vi "lua_monitor.vi"(11 "Lua for LabVIEW.lvlib:Lua.lvclass":refnum<class "Lua.lvclass">) -> ()   [LabVIEW 2020, in "Lua for LabVIEW.lvlib" / "Lua.lvclass"]
uses:
  Lua.lvclass
  Lua.lvclass/Lua.ctl
  lib/lua.dll/lua.dll.lvlib
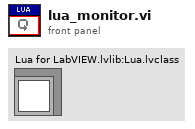
[diagram p1: front panel]
types:
  T1 = typedef "Lua for LabVIEW.lvlib/Lua.lvclass/lua_monitor_event.ctl" = enum16{"<null>", "terminate"}
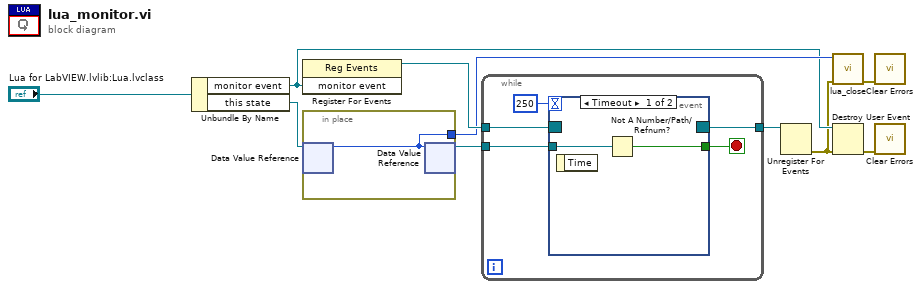
[diagram p0: block diagram]
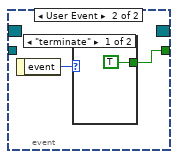
[diagram p2: hidden frame]
diagram:
  n1 = Unbundle By Name("Lua for LabVIEW.lvlib:Lua.lvclass") -> ("monitor event"=w2:refnum<user-event>, "this state"=w5:refnum<data-value>)
  n2 = register-events(w2) -> (reference out=w10:refnum<event-registration>)  [unwired: 2 in, 1 out]
  n3 = in-place {
    in-place-border: [w11] -> w3
    n4 = in-place-dvr #1(w5) -> (w11:u64)  [unwired: 1 out]
    n5 = in-place-dvr #1(w11) -> (w4:refnum<data-value>)  [unwired: 1 out]
  }
  n6 = while {
    tunnel: w4 -> [w14]
    tunnel: w10 -> [w16]
    tunnel: [w12] -> w8
    stop <- w13 stop-if-true
    n7 = event shown="[0] Timeout" {
      selector: w16 -> [_ _]
      dyn-events: [_ _] -> w12
      timeout: 250 -> [_ _]
      tunnel: w14 -> [w18 _]
      tunnel: [w17 w19] -> w13
      event Timeout {
        n8 = event-data() -> ()  [unwired: 1 in, 1 out]
        n9 = Not A Number/Path/Refnum?(number/path/refnum=w18) -> (NaN/Path/Refnum?=w17:bool)
      }
      event User Event {
        n10 = event-data() -> ("event"=w20:T1)  [unwired: 1 in]
        n11 = case shown="\"terminate\"" w20 {
          tunnel: [TRUE _] -> w19
          frame "terminate" {
          }
          frame Default {
          }
        }
      }
    }
  }
  n12 = Unregister For Events(event registration refnum=w8) -> (error out=w1:errorcluster)  [unwired: 1 in]
  n13 = call "lua_close.vi"("error in (no error)"=w1, "lua_state_p"=w3) -> ("error out"=w9:errorcluster)  [unwired: 9 in]
  n14 = Destroy User Event(user event=w2, error in=w1) -> (error out=w7:errorcluster)
  n15 = call <vilib>:"Clear Errors.vi"("error in (no error)"=w9) -> ()  [unwired: 5 in, 2 out]
  n16 = call <vilib>:"Clear Errors.vi"("error in (no error)"=w7) -> ()  [unwired: 5 in, 2 out]
